vi "parse CSV file for tags.vi"() -> (0 "create input tags?":bool, 1 "create output tags?":bool, 2 "create channels?":bool, 3 "tags":T1[](array[typedef]), 5 "outputs?":bool[](array[boolean]))   [LabVIEW 2013, in "EIP Tags editor node.lvclass"]
uses:
  EIP Tags editor node.lvclass
  configuration/eip tag definition.ctl
  configuration/eip tag types.ctl
  configuration/EIP Tags Configuration.lvclass
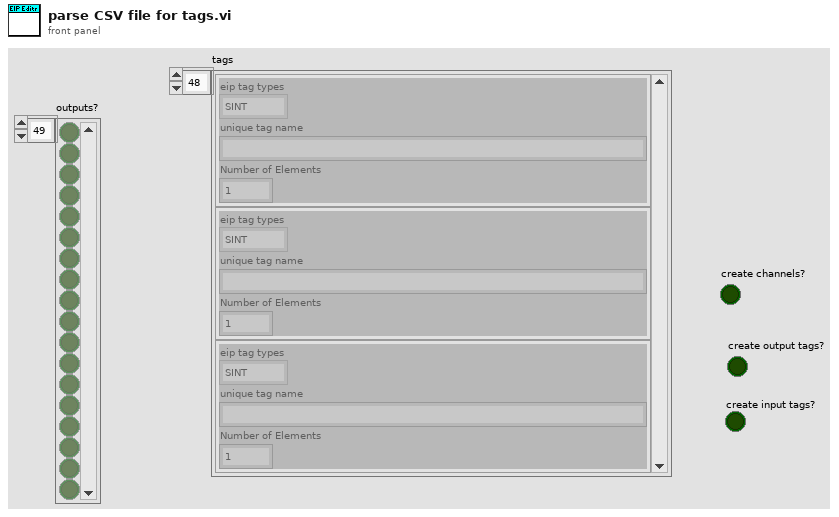
[diagram p1: front panel]
types:
  T1 = typedef "EIP Tags Configuration.lvclass/eip tag definition.ctl" = cluster{"eip tag types":T2, "unique tag name":string, "Number of Elements":u32}
  T2 = typedef "EIP Tags Configuration.lvclass/eip tag types.ctl" = enum16{"SINT", "INT", "DINT", "REAL", "BOOL", "STRING"}
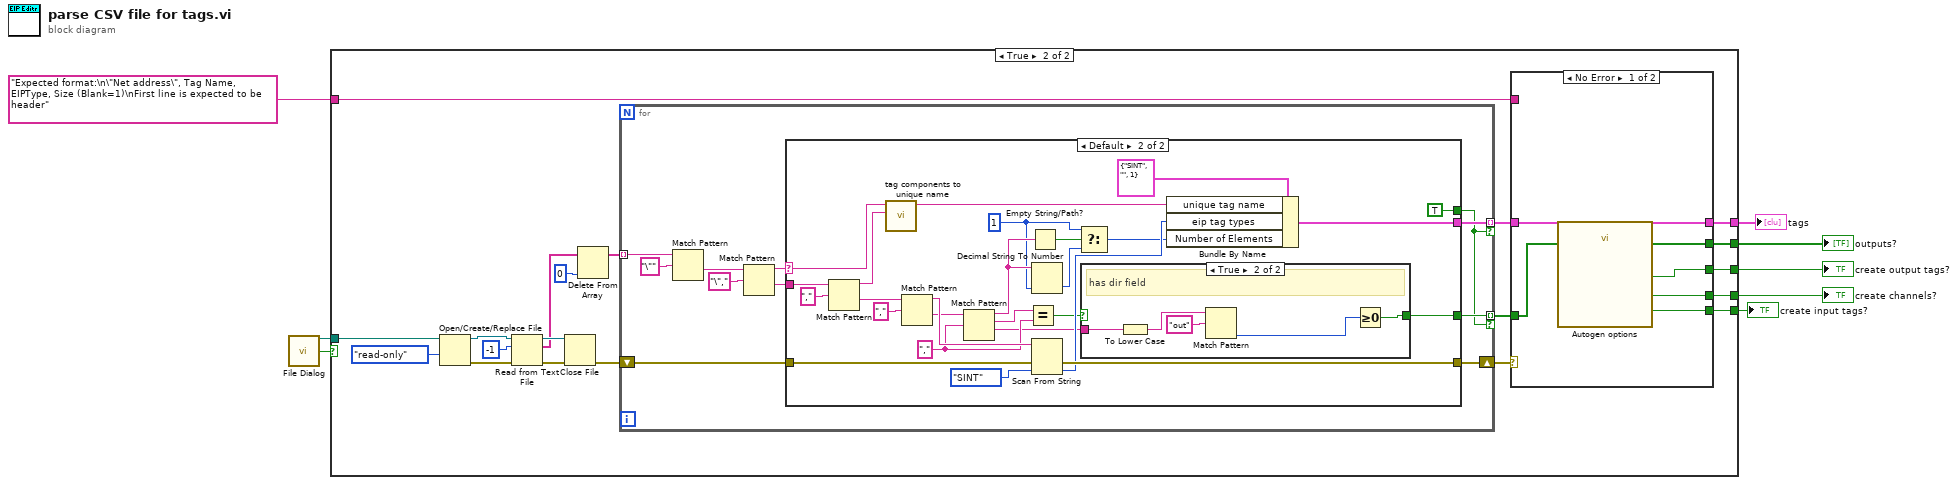
[diagram p0: block diagram]
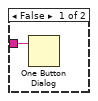
[diagram p2: hidden frame]
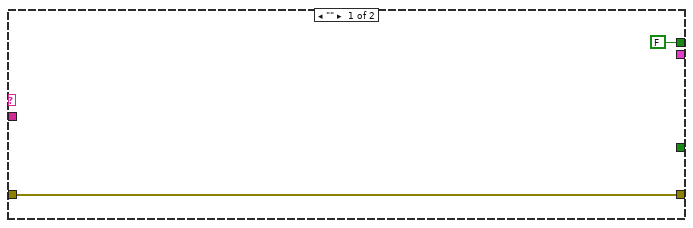
[diagram p3: hidden frame]
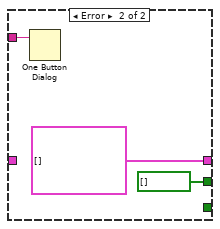
[diagram p5: hidden frame]
diagram:
  n1 = call "File Dialog"() -> ("selected path"=w4:path, "exists"=w5:bool)  [unwired: 12 in, 2 out]
  n2 = case shown="True" w5 {
    tunnel: [_ w29] -> w8
    tunnel: [_ w28] -> w7
    tunnel: [_ w27] -> w6
    tunnel: w4 -> [_ w24]
    tunnel: "Expected format:\n\"Net address\", Tag Name, EIPType, Size (Blank=1)\nFirst line is expected to be header" ("message") -> [w9 w26]
    tunnel: [_ w11] -> w2
    tunnel: [_ w10] -> w1
    frame False {
      n3 = One Button Dialog(message=w9) -> ()  [unwired: 1 in, 1 out]
    }
    frame True {
      n4 = Open/Create/Replace File(file path (use dialog)=w24, access (0:read/write)=enum16{"read/write", "read-only", "write-only"}."read-only") -> (refnum out=w22:refnum<file>, error out=w23:errorcluster)  [unwired: 4 in, 1 out]
      n5 = Read from Text File(file (use dialog)=w22, count=-1, error in=w23) -> (refnum out=w20:refnum<file>, text=w16:string[], error out=w19:errorcluster)  [unwired: 1 in, 1 out]
      n6 = Close File(refnum=w20, error in=w19) -> (error out=w18:errorcluster)  [unwired: 1 out]
      n7 = Delete From Array(array=w16, index=0) -> (array with subset deleted=w15:string[])  [unwired: 1 in, 1 out]
      n8 = for {
        shift-right: [w33] -> w14
        shift-left: w18 -> [w34]
        tunnel: w15 -> [w39] mode=indexing
        tunnel: [w40] -> w13 mode=indexing if=w30
        tunnel: [w31] -> w12 mode=indexing if=w30
        n9 = Match Pattern(string=w39, regular expression="\"") -> (after substring=w37:string)  [unwired: 1 in, 3 out]
        n10 = Match Pattern(string=w37, regular expression="\",") -> (before substring=w32:string, after substring=w35:string)  [unwired: 1 in, 2 out]
        n11 = case shown="Default" w32 {
          selector: w32 -> [_ w55]
          tunnel: [_ w67] -> w40
          tunnel: w35 -> [_ w65]
          tunnel: w34 -> [w41 w60]
          tunnel: [w41 w59] -> w33
          tunnel: [FALSE TRUE] -> w30
          tunnel: [_ w43] -> w31
          frame "" {
          }
          frame Default {
            w51 = "," ("regular expression")
            w46 = u32 1 ("Number of Elements")
            n12 = Match Pattern(string=w65, regular expression=",") -> (before substring=w61:string, after substring=w63:string)  [unwired: 1 in, 2 out]
            n13 = call "tag components to unique name.vi"("Tag Name"=w61, "Network Path"=w55) -> ("unique name"=w66:string)  [unwired: 9 in]
            n14 = Match Pattern(string=w63, regular expression=",") -> (before substring=w58:string, after substring=w53:string)  [unwired: 1 in, 2 out]
            n15 = Match Pattern(string=w53, regular expression=w51) -> (before substring=w47:string, match substring=w52:string, after substring=w49:string)  [unwired: 1 in, 1 out]
            n16 = Equal?(x=w52, y=w51) -> (x = y?=w50:bool)
            n17 = Empty String/Path?(string/path=w47) -> (empty?=w48:bool)
            n18 = Decimal String To Number(string=w47, default (0L)=w46) -> (number=w45:u32)  [unwired: 1 in, 1 out]
            n19 = Scan From String(input string=w58, error in=w60, default 1=eip_tag_types."SINT" ("eip tag types")) -> (error out=w59:errorcluster, output 1=w56:T2)  [unwired: 2 in, 2 out]
            n20 = Select(t=w46, s=w48, f=w45) -> (s? t:f=w44:u32)
            n21 = case shown="True" w50 {
              selector: w50 -> [w69 _]
              tunnel: w49 -> [_ w74]
              tunnel: [w69 w70] -> w43
              frame False {
                # "f=input, a safe default"
                # "no dir"
              }
              frame True {
                # "has dir field"
                n22 = To Lower Case(string=w74) -> (all lower case string=w73:string)
                n23 = Match Pattern(string=w73, regular expression="out") -> (offset past match=w71:i32)  [unwired: 1 in, 3 out]
                n24 = Greater Or Equal To 0?(x=w71) -> (x >= 0?=w70:bool)
              }
            }
            n25 = Bundle By Name(cluster=T1 {"eip tag types"=enum."SINT", "unique tag name"="", "Number of Elements"=1} ("tag spec"), "unique tag name"=w66, "eip tag types"=w56, "Number of Elements"=w44) -> (w67:T1)
          }
        }
      }
      n26 = case shown="No Error" w14 {
        tunnel: [w79 _] -> w29
        tunnel: [w78 _] -> w28
        tunnel: [w77 T1[] [] ("tags 2")] -> w27
        tunnel: w26 -> [_ w81]
        tunnel: w13 -> [w77 _]
        tunnel: w12 -> [w76 _]
        tunnel: [w76 bool[] []] -> w11
        tunnel: [w75 _] -> w10
        frame No Error {
          n27 = call "Autogen options"() -> ("Map Input Channels to Tags"=w75:bool, "Map Output Channels to Tags"=w78:bool, "Create Channels"=w79:bool)  [unwired: 15 in, 2 out]
        }
        frame Error {
          n28 = One Button Dialog(message=w81) -> ()  [unwired: 1 in, 1 out]
        }
      }
    }
  }
  "tags" <- w6
  "create channels?" <- w8
  "create output tags?" <- w7
  "outputs?" <- w2
  "create input tags?" <- w1
